vi "Write Running.vi"(8 "error in (no error)":errorcluster, 10 "Running":bool, 11 "Sequence Executor in":refnum<class "Sequence Executor.lvclass">) -> (0 "error out":errorcluster, 3 "Sequence Executor out":refnum<class "Sequence Executor.lvclass">)   [LabVIEW 2026, in "Sequence Executor.lvclass"]
doc: "Writes one field of this class's private data. Generated by lvai_create_accessors from the class private data control."
uses:
  Sequence Executor.lvclass
  Sequence Executor.lvclass/Sequence Executor.ctl
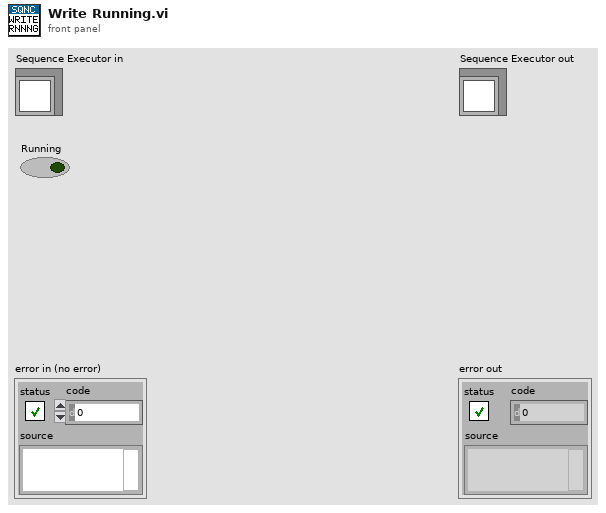
[diagram p1: front panel]
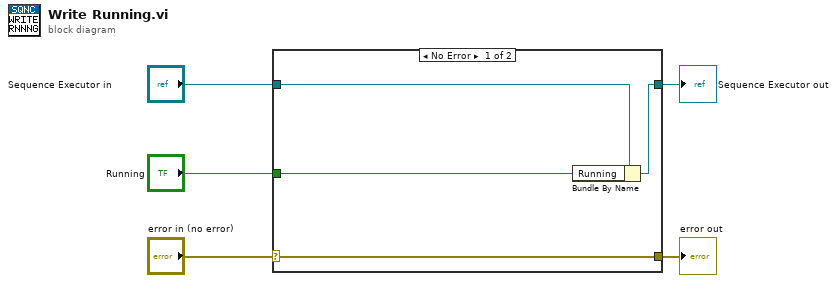
[diagram p0: block diagram]
diagram:
  n1 = case shown="No Error" "error in (no error)" {
    selector: "error in (no error)" -> [w9 w10]
    tunnel: [w9 w10] -> w4
    tunnel: [w7 w11] -> w2
    tunnel: "Sequence Executor in" -> [w8 w11]
    tunnel: "Running" -> [w6 _]
    frame No Error {
      n2 = Bundle By Name(cluster=w8, "Running"=w6) -> (w7:refnum<class "Sequence Executor.lvclass">)
    }
    frame Error {
    }
  }
  "error out" <- w4
  "Sequence Executor out" <- w2
